vi "permutation.vi"(11 "R":dbl) -> (10 "Output":dbl)   [LabVIEW 2018]
panel:
  in  "N":dbl
  # "Permuation"
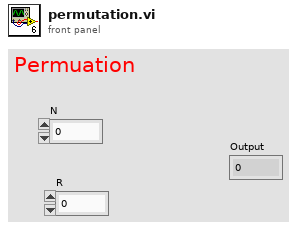
[diagram p1: front panel]
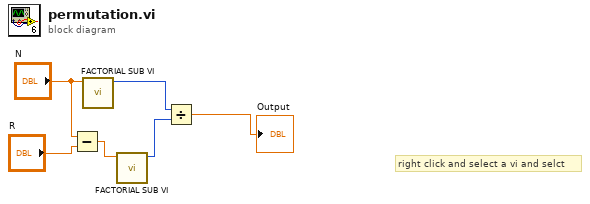
[diagram p0: block diagram]
diagram:
  # "right click and select a vi and selct"
  n1 = Subtract(x="N", y="R") -> (x-y=w4:dbl)
  n2 = call "FACTORIAL SUB VI.vi"("N"="N") -> ("x*y"=w3:i32)  [unwired: 10 in]
  n3 = call "FACTORIAL SUB VI.vi"("N"=w4) -> ("x*y"=w2:i32)  [unwired: 10 in]
  n4 = Divide(x=w3, y=w2) -> (x/y=→"Output":dbl)
